vi "Caller C1.vi"(0 "x":dbl, 11 "error in":errorcluster) -> (4 "y":dbl, 15 "error out":errorcluster)   [LabVIEW 2026]
doc: "Calls Target C1.vi once, to see whether LabVIEW inlines it."
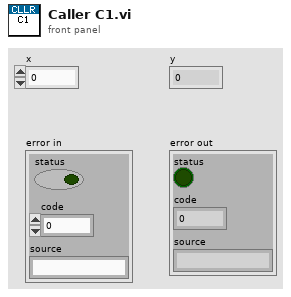
[diagram p1: front panel]
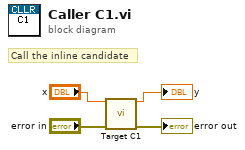
[diagram p0: block diagram]
diagram:
  # "Call the inline candidate"
  n1 = call "Target C1.vi"("x"="x", "error in"="error in") -> ("x times two"=→"y":dbl, "error out"=→"error out":errorcluster)  [unwired: 12 in]
